vi "Display Data.vi"(8 "error in (no error)":errorcluster, 9 "Test Data":cluster{"Best Linear Fit":dbl[], "Y":dbl[]}[](array[cluster]), 10 "XY Plot":refnum<vi>, 11 "3way Lap in":refnum<class "3way Lap.lvclass">) -> (0 "error out":errorcluster, 3 "3way Lap out":refnum<class "3way Lap.lvclass">)   [LabVIEW 2025, in "Flow Grind.lvlib" / "3way Lap.lvclass"]
uses:
  3way Lap.lvclass
  3way Lap.lvclass/3way Lap.ctl
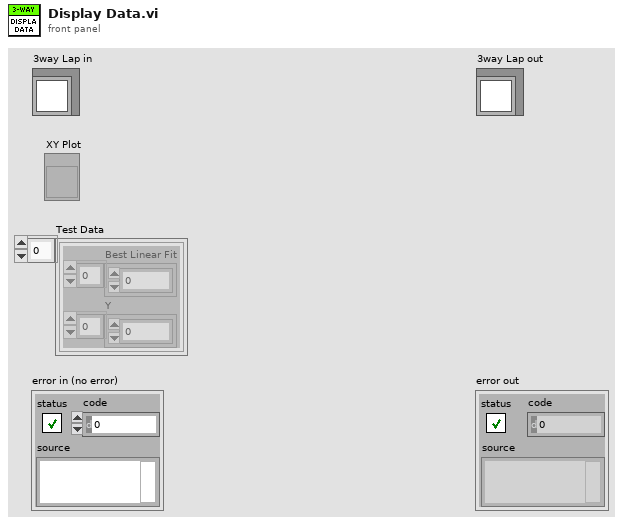
[diagram p1: front panel]
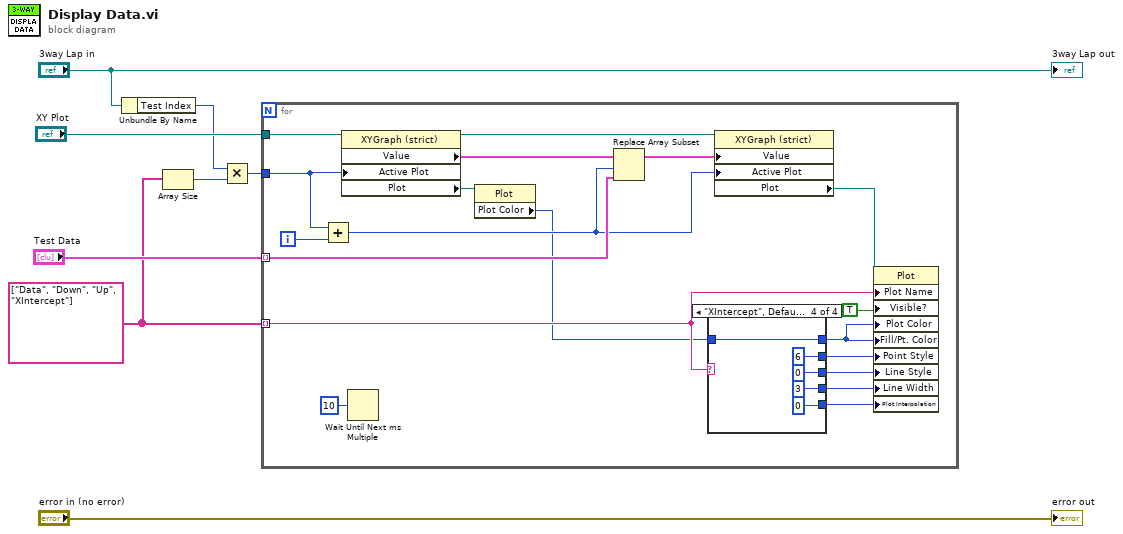
[diagram p0: block diagram]
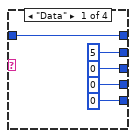
[diagram p2: hidden frame]
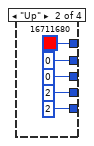
[diagram p3: hidden frame]
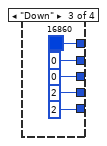
[diagram p4: hidden frame]
diagram:
  w3 = string[] ["Data", "Down", "Up", "XIntercept"]
  n1 = Unbundle By Name("3way Lap in") -> ("Test Index"=w4:u32)
  n2 = Array Size(array=w3) -> (size(s)=w2:i32)
  n3 = Multiply(x=w4, y=w2) -> (x*y=w1:u32)
  n4 = for {
    tunnel: "Test Data" -> [w27] mode=indexing
    tunnel: w3 -> [w15] mode=indexing
    tunnel: "XY Plot" -> [w19]
    tunnel: w1 -> [w9]
    i -> [w11]
    n5 = Add(x=w9, y=w11) -> (x+y=w14:u32)
    n6 = property class="XYGraph (strict)"(reference=w19, "Active Plot"=w9) -> (reference out=w20:refnum<vi>, "Value"=w21:cluster{dbl[], dbl[]}[], "Plot"=w13:refnum<vi>)  [unwired: 1 in, 1 out]
    n7 = Wait Until Next ms Multiple(millisecond multiple=u32 10) -> ()  [unwired: 1 out]
    n8 = property class="Plot"(reference=w13) -> ("Plot Color"=w12:u32)  [unwired: 1 in, 2 out]
    n9 = Replace Array Subset(array=w21, new element=w27, index=w14) -> (w18:cluster{dbl[], dbl[]}[])
    n10 = case shown="\"XIntercept\", Default" w15 {
      tunnel: [w28 u32 16711680 ("Plot.Plot Color") u32 16860 ("Plot.Plot Color") w43] -> w22
      tunnel: [u8 5 ("Plot.Point Style") u8 0 ("Plot.Point Style") u8 0 ("Plot.Point Style") u8 6 ("Plot.Point Style")] -> w26
      tunnel: [u8 0 ("Plot.Line Style") u8 0 ("Plot.Line Style") u8 0 ("Plot.Line Style") u8 0 ("Plot.Line Style")] -> w25
      tunnel: [u8 0 ("Plot.Line Width") u8 2 ("Plot.Line Width") u8 2 ("Plot.Line Width") u8 3 ("Plot.Line Width")] -> w24
      tunnel: [u8 0 ("Plot Interpolation") u8 2 ("Plot Interpolation") u8 2 ("Plot Interpolation") u8 0 ("Plot Interpolation")] -> w23
      tunnel: w12 -> [w28 _ _ w43]
      frame "Data" {
      }
      frame "Up" {
      }
      frame "Down" {
      }
      frame "XIntercept", Default {
      }
    }
    n11 = property class="XYGraph (strict)"(reference=w20, "Value"=w18, "Active Plot"=w14) -> ("Plot"=w17:refnum<vi>)  [unwired: 1 in, 2 out]
    n12 = property class="Plot"(reference=w17, "Plot Name"=w15, "Visible?"=TRUE ("Visible"), "Plot Color"=w22, "Fill/Pt. Color"=w22, "Point Style"=w26, "Line Style"=w25, "Line Width"=w24, "Plot Interpolation"=w23) -> ()  [unwired: 1 in, 2 out]
  }
  "error out" <- "error in (no error)"
  "3way Lap out" <- "3way Lap in"
